vi "recall Param.vi"(8 "error in (no error)":errorcluster caption="에러 입력(에러 없음)", 10 "Recall Name":string, 11 "NR 입력":refnum<class "NR.lvclass">) -> (0 "error out":errorcluster caption="에러 출력", 3 "NR 출력":refnum<class "NR.lvclass">)   [LabVIEW 2023, in "ANRITSU Call Box.lvlib" / "NR.lvclass"]
uses:
  NR.lvclass
  <vilib>/regexp/Match Regular Expression.xnode
  NR.lvclass/NR.ctl
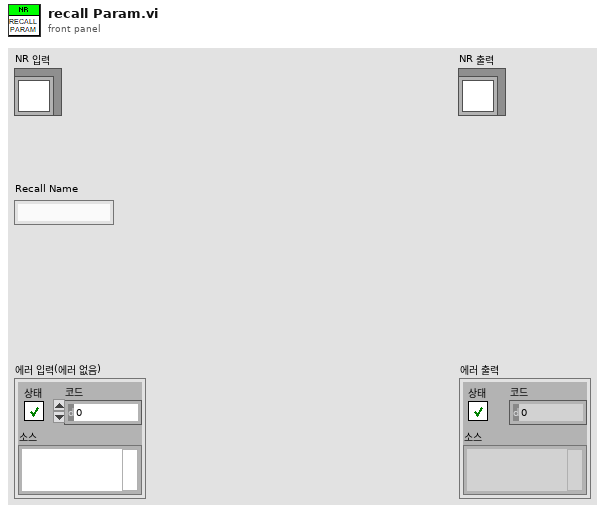
[diagram p1: front panel]
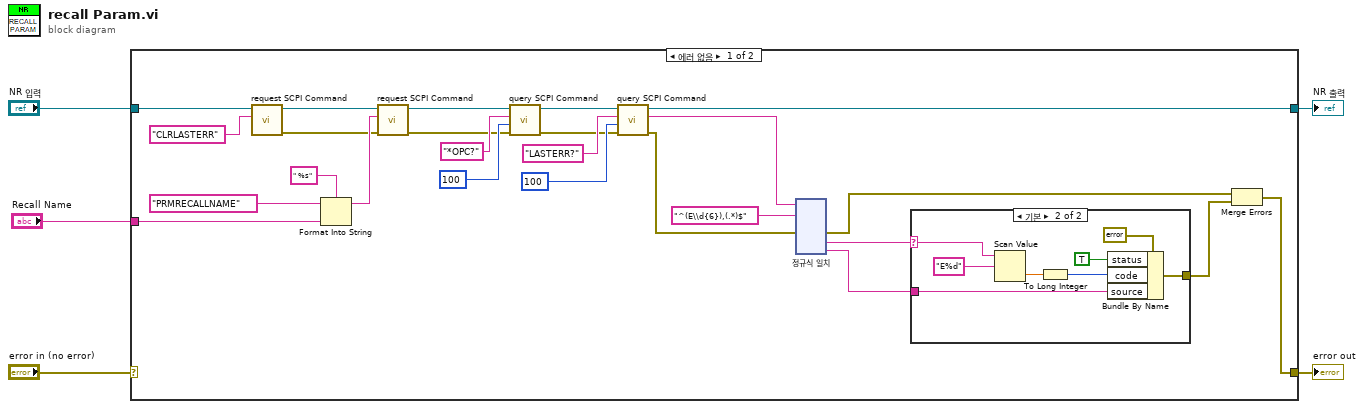
[diagram p0: block diagram]
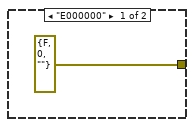
[diagram p2: hidden frame]
diagram:
  n1 = case shown="에러 없음" "error in (no error)" {
    selector: "error in (no error)" -> [_ w161]
    tunnel: [w6 w161] -> w4
    tunnel: [w19 w160] -> w2
    tunnel: "NR 입력" -> [w17 w160]
    tunnel: "Recall Name" -> [w28 _]
    frame No Error {
      n2 = call "request SCPI Command.vi"("SCPI Command"="CLRLASTERR" ("write buffer"), "NR in"=w17) -> ("error out"=w15:errorcluster, "NR out"=w16:refnum<class "NR.lvclass">)  [unwired: 8 in]
      n3 = Format Into String(format string=" %s", initial string="PRMRECALLNAME" ("write buffer"), w28) -> (resulting string=w27:string)  [unwired: 1 in, 1 out]
      n4 = call "request SCPI Command.vi"("error in (no error)"=w15, "SCPI Command"=w27, "NR in"=w16) -> ("error out"=w23:errorcluster, "NR out"=w24:refnum<class "NR.lvclass">)  [unwired: 7 in]
      n5 = call "query SCPI Command.vi"("error in (no error)"=w23, "Read Buffer Length"=u32 100, "SCPI Command"="*OPC?", "NR in"=w24) -> ("error out"=w18:errorcluster, "NR out"=w20:refnum<class "NR.lvclass">)  [unwired: 5 in, 1 out]
      n6 = call "query SCPI Command.vi"("error in (no error)"=w18, "Read Buffer Length"=u32 100, "SCPI Command"="LASTERR?", "NR in"=w20) -> ("error out"=w12:errorcluster, "Read Buffer String"=w11:string, "NR out"=w19:refnum<class "NR.lvclass">)  [unwired: 5 in]
      n7 = xnode "정규식 일치"("입력 문자열"=w11, "정규식"="^(E\\d{6}),(.*)$", "에러 입력"=w12) -> ("에러 출력"=w8:errorcluster, "부분 일치 1"=w10:string, "부분 일치 2"=w9:string)  [unwired: 3 in, 4 out]
      n8 = case shown="기본" w10 {
        selector: w10 -> [_ w38]
        tunnel: w9 -> [_ w34]
        tunnel: [errorcluster {"status"=FALSE, "code"=0, "source"=""} ("에러 출력") w32] -> w7
        frame "E000000" {
        }
        frame Default {
          n9 = Scan Value(string=w38, format string="E%d" ("포맷 문자열")) -> (value=w36:dbl)  [unwired: 1 in, 1 out]
          n10 = To Long Integer(number=w36) -> (32bit integer=w35:i32)
          n11 = Bundle By Name(cluster=errorcluster {"status"=TRUE, "code"=0, "source"=""} ("에러 출력"), "status"=TRUE, "code"=w35, "source"=w34) -> (w32:errorcluster)
        }
      }
      n12 = Merge Errors(w8, w7) -> (w6:errorcluster)
    }
    frame Error {
    }
  }
  "error out" <- w4
  "NR 출력" <- w2
